vi "Create Volatus API.vi"(8 "error in (no error)":errorcluster, 11 "Volatus Core in":refnum<class "Volatus Core.lvclass">) -> (0 "error out":errorcluster, 3 "Volatus Core out":refnum<class "Volatus Core.lvclass">)   [LabVIEW 2020, in "Volatus.lvlib" / "Volatus Core.lvclass"]
uses:
  Volatus Core.lvclass
  C:/dev/lv20CE/relink/lv-volatus/Volatus/Module/Module.lvclass
  Volatus Core.lvclass/Volatus Core.ctl
  Module/Module.lvclass/Module.ctl
  VolatusAPI/VolatusAPI.lvclass
  Module/Module.lvclass
  VolatusConfig/Node/Node Config.lvclass
  VolatusConfig/Cluster/Cluster Config.lvclass
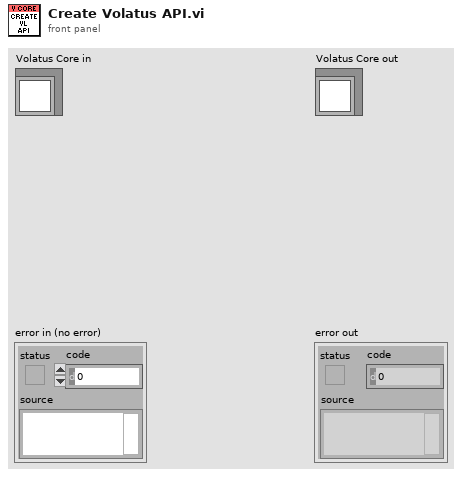
[diagram p1: front panel]
types:
  T1 = typedef "Volatus.lvlib/Target Info.ctl" = cluster{"ID":u32, "Type":T2}
  T2 = typedef "Volatus.lvlib/Target Type.ctl" = enum16{"Node", "Group"}
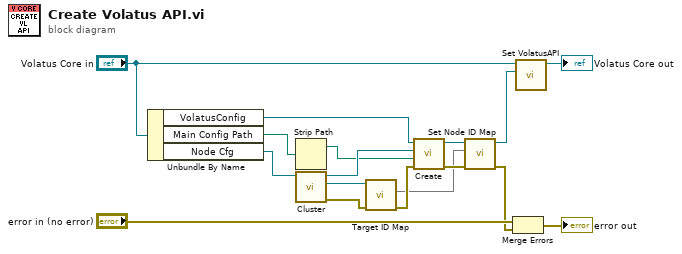
[diagram p0: block diagram]
diagram:
  n1 = Unbundle By Name("Volatus Core in") -> ("VolatusConfig"=w1:refnum<class "VolatusConfig.lvclass">, "Main Config Path"=w3:path, "Node Cfg"=w14:refnum<class "Node Config.lvclass">)
  n2 = Strip Path(path=w3) -> (stripped path=w2:path)  [unwired: 1 out]
  n3 = call "Cluster.vi"("Node in"=w14) -> ("error out"=w10:errorcluster, "Cluster"=w13:refnum<class "Cluster Config.lvclass">, "Node out"=w4:refnum<class "Node Config.lvclass">)  [unwired: 8 in]
  n4 = call "Target ID Map.vi"("error in (no error)"=w10, "Cluster in"=w13) -> ("error out"=w11:errorcluster, "Target ID Map"=w8:map{string, T1})  [unwired: 7 in, 1 out]
  n5 = call "Create.vi"("error in (no error)"=w11, "Config Folder"=w2, "Node Config"=w4, "Volatus Config"=w1) -> ("error out"=w9:errorcluster, "VolatusAPI out"=w12:refnum<class "VolatusAPI.lvclass">)  [unwired: 6 in]
  n6 = call "Set Node ID Map.vi"("error in (no error)"=w9, "Target IDs"=w8, "VolatusAPI in"=w12) -> ("error out"=w5:errorcluster, "VolatusAPI out"=w7:refnum<class "VolatusAPI.lvclass">)  [unwired: 7 in]
  n7 = Merge Errors("error in (no error)", w5) -> (→"error out":errorcluster)
  n8 = call "Set VolatusAPI.vi"("VolatusAPI"=w7, "Module in"="Volatus Core in") -> ("Module out"=→"Volatus Core out":refnum<class "Volatus Core.lvclass">)  [unwired: 9 in]
